vi "DrawSubMenuItems.vi"(7 "Collection in":refnum<class "Collection.lvclass">, 8 "error in (no error)":errorcluster, 9 "Coords":T2, 10 "Tag":string, 11 "Menu in":refnum<class "Menu.lvclass">) -> (0 "error out":errorcluster, 1 "SubMenu":bool, 2 "SelectedArea":T1, 3 "Menu out":refnum<class "Menu.lvclass">, 4 "SelectedItemTag":string, 5 "Collection out":refnum<class "Collection.lvclass">, 6 "GlobalArea":T1)   [LabVIEW 2021, in "Menu.lvlib" / "Menu.lvclass"]
uses:
  Menu.lvclass
  <vilib>/Utility/miscctls.llb/LVPoint32TypeDef.ctl
  Picture2D/src/Collection/Collection.lvclass
  C:/GitHub/Picture2D/src/IDrawable/IDrawable.lvclass
  Picture2D/src/Text/Text.lvclass
  C:/GitHub/Picture2D/src/Picture2D/Picture2D.lvclass
  C:/GitHub/Picture2D/src/Shape/Shape.lvclass
  Picture2D/src/Rectangle/Rectangle.lvclass
  C:/GitHub/Picture2D/src/Polygone/Polygone.lvclass
  Picture2D/src/Point/Point.lvclass
  Picture2D/src/PointSpecialized/PointSpecialized.lvclass
  C:/GitHub/Picture2D/src/Point/Point.lvclass
  Picture2D/src/PointSpecialized/PointSpecialized.lvclass/PointSpecialized.ctl
  Picture2D/src/PointSpecialized/SetColor.vi
  Picture2D/src/Picture/Image.lvclass
  GetFont.vi
  GetDesiredFont.vi
  Picture2D/src/Font/Font.lvclass
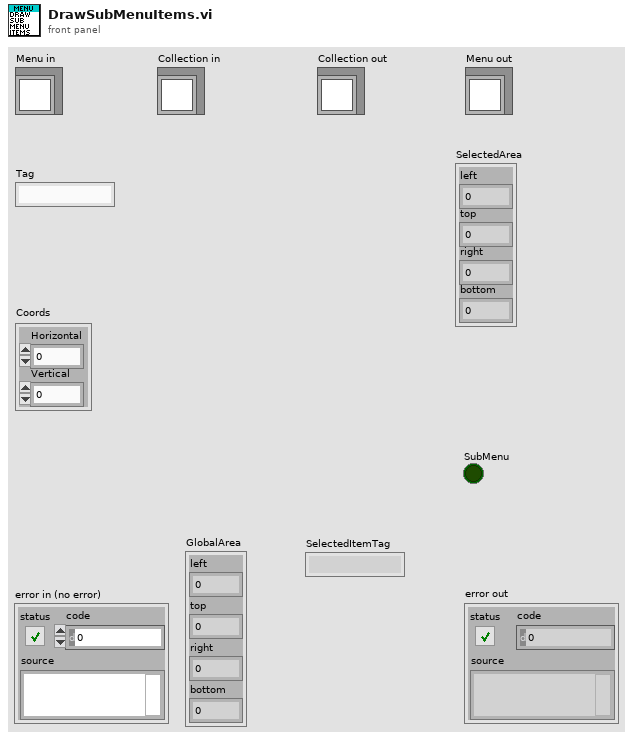
[diagram p1: front panel]
types:
  T1 = cluster{"left":i16, "top":i16, "right":i16, "bottom":i16}
  T2 = typedef "LVPoint32TypeDef.ctl" = cluster{"Horizontal":i32, "Vertical":i32}
  T3 = typedef "Menu.lvlib/Menu.lvclass/MenuItems.ctl" = cluster{"Item Name":string, "Short Cut":T4, "Checked":bool, "Enable":bool, "After item":string, "Item Tags":string[], "Item Names":string[], "Picture":refnum<class "Image.lvclass">, "Hilite Picture":refnum<class "Image.lvclass">, "Displayed":bool}
  T4 = typedef "LVMenuShortCut.ctl" = cluster{"Include Shift Key?":bool, "Include Ctrl Key?":bool, "Shortcut Key":string}
  T5 = typedef "Menu.lvlib/Menu.lvclass/MenuColors.ctl" = cluster{"Text":refnum<class "Color.lvclass">, "HiliteText":refnum<class "Color.lvclass">, "Background":refnum<class "Color.lvclass">, "BorderColor":refnum<class "Color.lvclass">, "Hilite":refnum<class "Color.lvclass">}
  T6 = enum16{"User-specified Font", "Application Font", "System Font", "Dialog Font"}
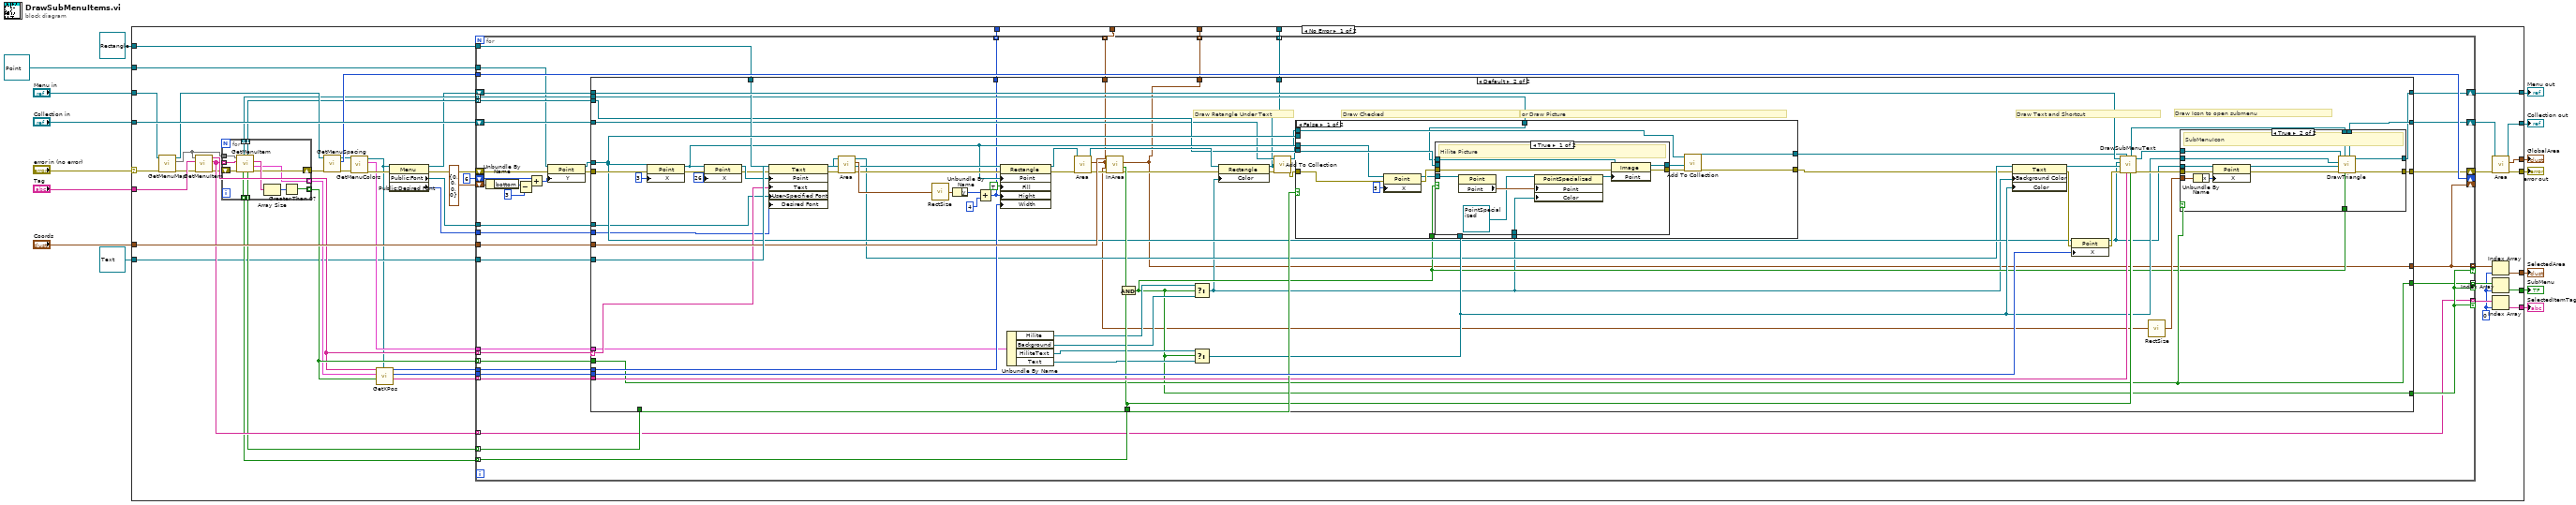
[diagram p0: block diagram]
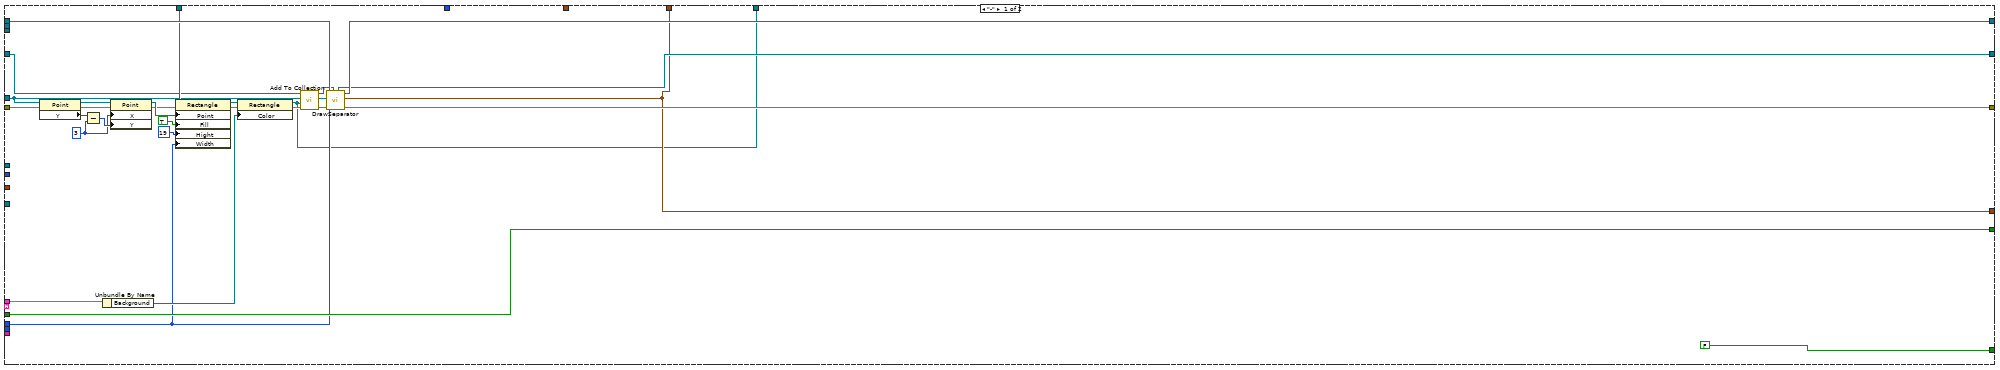
[diagram p2: hidden frame]
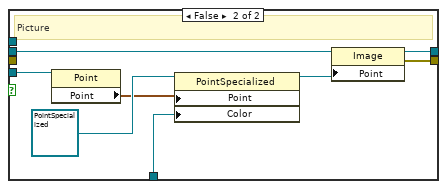
[diagram p3: hidden frame]
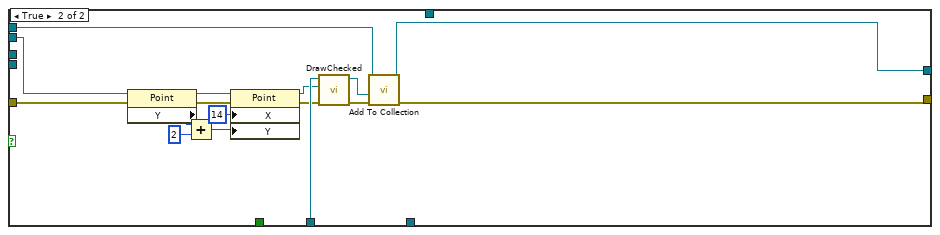
[diagram p4: hidden frame]
diagram:
  n1 = case shown="No Error" "error in (no error)" {
    selector: "error in (no error)" -> [w49 w279]
    tunnel: [w68 _] -> w15
    tunnel: [w66 _] -> w14
    tunnel: "Coords" -> [w62 _]
    tunnel: [w34 _] -> w12
    tunnel: [w55 _] -> w11
    tunnel: "Collection in" -> [w53 w280]
    tunnel: [w29 w280] -> w9
    tunnel: "Menu in" -> [w51 w281]
    tunnel: "Tag" -> [w47 _]
    tunnel: [w40 w279] -> w5
    tunnel: [w30 w281] -> w4
    tunnel: refnum<class "Text.lvclass"> refnum ("Picture2D.lvlib:Text") -> [w27 _]
    tunnel: refnum<class "Point.lvclass"> refnum ("PointSpecialized") -> [w26 _]
    tunnel: refnum<class "Rectangle.lvclass"> refnum ("Rectangle") -> [w25 _]
    tunnel: [w19 _] -> _
    tunnel: [w18 _] -> _
    tunnel: [w17 _] -> _
    tunnel: [w16 _] -> _
    frame No Error {
      w56 = 0 ("index")
      n2 = call "GetMenuMap.vi"("error in (no error)"=w49, "Menu in"=w51) -> ("error out"=w44:errorcluster, "MenuMap"=w48:map{string, T3}, "Menu out"=w50:refnum<class "Menu.lvclass">)  [unwired: 7 in]
      n3 = call "GetMenuItem.vi"("error in (no error)"=w44, "Tag"=w47, "MenuMap"=w48) -> ("error out"=w43:errorcluster, "Item Tags"=w45:string[], "Item Names"=w46:string[])  [unwired: 1 in, 5 out]
      n4 = for {
        tunnel: w48 -> [w278]
        tunnel: w45 -> [w277] mode=indexing
        tunnel: [w274] -> w54 mode=indexing
        shift-right: [w272] -> w42
        shift-left: w43 -> [w273]
        tunnel: [w271] -> w39 mode=indexing
        tunnel: [w270] -> w38 mode=indexing
        tunnel: [w269] -> w37 mode=indexing
        tunnel: [w268] -> w36 mode=indexing
        tunnel: [w267] -> w35 mode=indexing
        n5 = call "GetMenuItem.vi"("error in (no error)"=w273, "Tag"=w277, "MenuMap"=w278) -> ("error out"=w272:errorcluster, "Short Cut"=w271:T4, "Item Tags"=w276:string[], "Checked"=w270:bool, "Picture"=w268:refnum<class "Image.lvclass">, "Enable"=w269:bool, "Hilite Picture"=w267:refnum<class "Image.lvclass">)  [unwired: 1 in, 1 out]
        n6 = Array Size(array=w276) -> (size(s)=w275:i32)
        n7 = Greater Than 0?(x=w275) -> (x > 0?=w274:bool)
      }
      n8 = call "GetMenuSpacing.vi"("error in (no error)"=w42, "Menu in"=w50) -> ("error out"=w41:errorcluster, "MenuSpacing"=w52:i32, "Menu out"=w33:refnum<class "Menu.lvclass">)  [unwired: 7 in]
      n9 = call "GetMenuColors.vi"("error in (no error)"=w41, "Menu in"=w33) -> ("error out"=w31:errorcluster, "MenuColors"=w28:T5, "Menu out"=w20:refnum<class "Menu.lvclass">)  [unwired: 7 in]
      n10 = call "GetXPos.vi"("Menu"=w20, "SubMenu"=w54, "Array"=w39, "Item Names"=w46) -> ("ShortCut Text"=w59:string[], "Start ShortCut"=w60:i16, "Total X"=w61:i16)  [unwired: 5 in]
      n11 = property class="Menu"(reference=w20, error in=w31) -> (reference out=w23:refnum<class "Menu.lvclass">, error out=w24:errorcluster, "Public:Font"=w22:refnum<class "Font.lvclass">, "Public:Desired Font"=w21:T6)
      n12 = for {
        tunnel: w46 -> [w101] mode=indexing
        shift-right: [w98] -> w58
        shift-left: w53 -> [w99]
        shift-right: [w100] -> _
        shift-left: T1 {"left"=0, "top"=0, "right"=0, "bottom"=0} ("Area out") -> [w106]
        tunnel: w62 -> [w103]
        shift-right: [w102] -> _
        shift-left: i16 6 ("Spacing") -> [w104]
        tunnel: w52 -> [w102]
        tunnel: [w83] -> w65 mode=indexing if=w93
        tunnel: [w100] -> w67 mode=indexing if=w93
        tunnel: w45 -> [w83] mode=indexing
        tunnel: w61 -> [w97]
        tunnel: w60 -> [w96]
        tunnel: w59 -> [w95] mode=indexing
        tunnel: w54 -> [w94] mode=indexing
        tunnel: [w84] -> w57 mode=indexing if=w93
        tunnel: w38 -> [w90] mode=indexing
        tunnel: w37 -> [w85] mode=indexing
        tunnel: w36 -> [w91] mode=indexing
        tunnel: w35 -> [w89] mode=indexing
        shift-right: [w88] -> w32
        shift-left: w24 -> [w87]
        shift-right: [w76] -> w30
        shift-left: w23 -> [w86]
        tunnel: w28 -> [w82]
        tunnel: w27 -> [w81]
        tunnel: w26 -> [w80]
        tunnel: w25 -> [w79]
        tunnel: w22 -> [w78]
        tunnel: w21 -> [w77]
        tunnel: [w75] -> w19 mode=indexing
        tunnel: [w74] -> w18 mode=indexing
        tunnel: [w73] -> w17 mode=indexing
        tunnel: [w72] -> w16 mode=indexing
        n13 = Unbundle By Name(w106) -> ("bottom"=w71:i16)
        n14 = Subtract(x=w71, y=i16 3) -> (x-y=w70:i16)
        n15 = Add(x=w104, y=w70) -> (x+y=w105:i32)
        n16 = property class="Point"(reference=w80, error in=w87, "Y"=w105) -> (reference out=w107:refnum<class "Point.lvclass">, error out=w92:errorcluster)
        n17 = case shown="Default" w101 {
          selector: w101 -> [_ w195]
          tunnel: w107 -> [w119 w173]
          tunnel: w103 -> [_ w198]
          tunnel: w81 -> [_ w203]
          tunnel: [w109 w138] -> w100
          tunnel: [FALSE ("InArea") w150] -> w93
          tunnel: w99 -> [w122 w145]
          tunnel: [w110 w158] -> w98
          tunnel: w97 -> [w123 w196]
          tunnel: w96 -> [_ w194]
          tunnel: w95 -> [_ w182]
          tunnel: w94 -> [w135 w180]
          tunnel: [w135 w180] -> w84
          tunnel: w92 -> [w111 w192]
          tunnel: w91 -> [_ w149]
          tunnel: w90 -> [_ w187]
          tunnel: w89 -> [_ w148]
          tunnel: [w134 w177] -> w88
          tunnel: w86 -> [w133 w184]
          tunnel: w85 -> [_ w181]
          tunnel: w82 -> [w126 w172]
          tunnel: w79 -> [w124 w167]
          tunnel: w78 -> [_ w156]
          tunnel: w77 -> [_ w162]
          tunnel: [w132 w157] -> w76
          tunnel: [_ w140] -> w75
          tunnel: [w109 w138] -> w74
          tunnel: [_ w139] -> w73
          tunnel: [w108 w137] -> w72
          frame "-" {
            w115 = i16 3 ("Point:x")
            n18 = property class="Point"(reference=w119, error in=w111) -> (reference out=w116:refnum<class "Point.lvclass">, error out=w114:errorcluster, "Y"=w118:i16)
            n19 = Subtract(x=w118, y=w115) -> (x-y=w117:i16)
            n20 = Unbundle By Name(w126) -> ("Background"=w125:refnum<class "Color.lvclass">)
            n21 = property class="Point"(reference=w116, error in=w114, "X"=w115, "Y"=w117) -> (reference out=w120:refnum<class "Point.lvclass">, error out=w113:errorcluster)
            n22 = property class="Rectangle"(reference=w124, error in=w113, "Point"=w120, "Fill"=TRUE, "Hight"=i16 19 ("x"), "Width"=w123) -> (reference out=w128:refnum<class "Rectangle.lvclass">, error out=w130:errorcluster)
            n23 = property class="Rectangle"(reference=w128, error in=w130, "Color"=w125) -> (reference out=w108:refnum<class "Rectangle.lvclass">, error out=w129:errorcluster)
            n24 = call-dynamic "Add To Collection.vi"("error in (no error)"=w129, "IDrawable"=w108, "Collection in"=w122) -> ("error out"=w112:errorcluster, "Collection out"=w121:refnum<class "Collection.lvclass">)  [unwired: 7 in]
            n25 = call "DrawSeparator.vi"("Collection in"=w121, "error in (no error)"=w112, "XPos"=w123, "Point"=w119, "Menu in"=w133) -> ("error out"=w134:errorcluster, "rect"=w109:T1, "Menu out"=w132:refnum<class "Menu.lvclass">, "Collection out"=w110:refnum<class "Collection.lvclass">)  [unwired: 3 in]
          }
          frame Default {
            # "Draw Retangle Under Text"
            # "Draw Checked"
            # "or Draw Picture"
            # "Draw Icon to open submenu"
            # "Draw Text and Shortcut"
            n26 = property class="Point"(reference=w173, error in=w192, "X"=i16 3 ("Point:x")) -> (reference out=w151:refnum<class "Point.lvclass">, error out=w166:errorcluster)
            n27 = property class="Point"(reference=w151, error in=w166, "X"=i16 26 ("Point:x")) -> (reference out=w202:refnum<class "Point.lvclass">, error out=w165:errorcluster)
            n28 = property class="Text"(reference=w203, error in=w165, "Point"=w202, "Text"=w195, "User-Specified Font"=w156, "Desired Font"=w162) -> (reference out=w155:refnum<class "Text.lvclass">, error out=w191:errorcluster)
            n29 = call-dynamic "Area.vi"("error in (no error)"=w191, "Text in"=w155) -> ("error out"=w190:errorcluster, "rect"=w197:T1, "Text out"=w154:refnum<class "Text.lvclass">)  [unwired: 7 in]
            n30 = call <vilib>:"RectSize.vi"("rect"=w197) -> ("point"=w199:cluster{"x":i16, "y":i16})
            n31 = Unbundle By Name(w199) -> ("y"=w153:i16)
            n32 = Add(x=w153, y=i16 4) -> (x+y=w140:i16)
            n33 = property class="Rectangle"(reference=w167, error in=w190, "Point"=w151, "Fill"=TRUE, "Hight"=w140, "Width"=w196) -> (reference out=w164:refnum<class "Rectangle.lvclass">, error out=w189:errorcluster)
            n34 = Unbundle By Name(w172) -> ("Hilite"=w168:refnum<class "Color.lvclass">, "Background"=w169:refnum<class "Color.lvclass">, "HiliteText"=w171:refnum<class "Color.lvclass">, "Text"=w170:refnum<class "Color.lvclass">)
            n35 = call-dynamic "Area.vi"("error in (no error)"=w189, "Rectangle in"=w164) -> ("error out"=w188:errorcluster, "rect"=w139:T1, "Rectangle out"=w163:refnum<class "Rectangle.lvclass">)  [unwired: 7 in]
            n36 = call "InArea.vi"("error in (no error)"=w188, "Area in"=w139, "Coords"=w198) -> ("error out"=w146:errorcluster, "InArea"=w186:bool, "Area out"=w138:T1)  [unwired: 6 in]
            n37 = Compound Arithmetic op=AND(w186, w181) -> (w150:bool)
            n38 = Select(t=w168, s=w150, f=w169) -> (s? t:f=w147:refnum<class "Color.lvclass">)
            n39 = Select(t=w171, s=w150, f=w170) -> (s? t:f=w174:refnum<class "Color.lvclass">)
            n40 = property class="Rectangle"(reference=w163, error in=w146, "Color"=w147) -> (reference out=w137:refnum<class "Rectangle.lvclass">, error out=w185:errorcluster)
            n41 = call-dynamic "Add To Collection.vi"("error in (no error)"=w185, "IDrawable"=w137, "Collection in"=w145) -> ("error out"=w142:errorcluster, "Collection out"=w144:refnum<class "Collection.lvclass">)  [unwired: 7 in]
            n42 = case shown="False" w187 {
              tunnel: w144 -> [w211 w250]
              tunnel: w142 -> [w213 w239]
              tunnel: w174 -> [_ w249]
              tunnel: w173 -> [_ w237]
              tunnel: w151 -> [w204 _]
              tunnel: w150 -> [w210 _]
              tunnel: w149 -> [w209 _]
              tunnel: w148 -> [w208 _]
              tunnel: w147 -> [w207 _]
              tunnel: [w205 w235] -> w141
              tunnel: [w206 w236] -> w143
              frame False {
                n43 = property class="Point"(reference=w204, error in=w213, "X"=i16 5 ("Point:x")) -> (reference out=w215:refnum<class "Point.lvclass">, error out=w217:errorcluster)
                n44 = case shown="True" w210 {
                  tunnel: w209 -> [_ w233]
                  tunnel: [w226 w234] -> w214
                  tunnel: w215 -> [w221 w231]
                  tunnel: w208 -> [w225 _]
                  tunnel: [w224 w232] -> w216
                  tunnel: w217 -> [w223 _]
                  tunnel: w207 -> [w218 w227]
                  frame True {
                    # "Hilite Picture"
                    n45 = property class="Point"(reference=w221) -> ("Point"=w222:cluster{"x":i16, "y":i16})  [unwired: 1 in, 2 out]
                    n46 = property class="PointSpecialized"(reference=refnum<class "PointSpecialized.lvclass"> refnum ("Picture2D.lvlib:PointSpecialized"), "Point"=w222, "Color"=w218) -> (reference out=w220:refnum<class "PointSpecialized.lvclass">)  [unwired: 1 in, 1 out]
                    n47 = property class="Image"(reference=w225, error in=w223, "Point"=w220) -> (reference out=w226:refnum<class "Image.lvclass">, error out=w224:errorcluster)
                  }
                  frame False {
                    # "Picture"
                    n48 = property class="Point"(reference=w231) -> ("Point"=w229:cluster{"x":i16, "y":i16})  [unwired: 1 in, 2 out]
                    n49 = property class="PointSpecialized"(reference=refnum<class "PointSpecialized.lvclass"> refnum ("Picture2D.lvlib:PointSpecialized"), "Point"=w229, "Color"=w227) -> (reference out=w228:refnum<class "PointSpecialized.lvclass">)  [unwired: 1 in, 1 out]
                    n50 = property class="Image"(reference=w233, "Point"=w228) -> (reference out=w234:refnum<class "Image.lvclass">, error out=w232:errorcluster)  [unwired: 1 in]
                  }
                }
                n51 = call-dynamic "Add To Collection.vi"("error in (no error)"=w216, "IDrawable"=w214, "Collection in"=w211) -> ("error out"=w205:errorcluster, "Collection out"=w206:refnum<class "Collection.lvclass">)  [unwired: 7 in]
              }
              frame True {
                n52 = property class="Point"(reference=w237, error in=w239) -> (reference out=w245:refnum<class "Point.lvclass">, error out=w238:errorcluster, "Y"=w246:i16)
                n53 = Add(x=w246, y=i16 2) -> (x+y=w247:i16)
                n54 = property class="Point"(reference=w245, error in=w238, "X"=i16 14 ("Point:x"), "Y"=w247) -> (reference out=w242:refnum<class "Point.lvclass">, error out=w241:errorcluster)
                n55 = call "DrawChecked.vi"("error in"=w241, "Point"=w242, "Color"=w249) -> ("error out"=w240:errorcluster, "Collection out"=w248:refnum<class "Collection.lvclass">)  [unwired: 7 in]
                n56 = call-dynamic "Add To Collection.vi"("error in (no error)"=w240, "IDrawable"=w248, "Collection in"=w250) -> ("error out"=w235:errorcluster, "Collection out"=w236:refnum<class "Collection.lvclass">)  [unwired: 7 in]
              }
            }
            n57 = property class="Text"(reference=w154, error in=w141, "Background Color"=w147, "Color"=w174) -> (reference out=w183:refnum<class "Text.lvclass">, error out=w176:errorcluster)
            n58 = property class="Point"(reference=w173, error in=w176, "X"=w194) -> (reference out=w160:refnum<class "Point.lvclass">, error out=w175:errorcluster)
            n59 = call "DrawSubMenuText.vi"("Enable"=w181, "ShortcutText"=w182, "Collection in"=w143, "error in (no error)"=w175, "Text"=w183, "InsertionPoint"=w160, "Menu in"=w184) -> ("error out"=w178:errorcluster, "Menu out"=w161:refnum<class "Menu.lvclass">, "Collection out"=w159:refnum<class "Collection.lvclass">)  [unwired: 2 in]
            n60 = call <vilib>:"RectSize.vi"("rect"=w139) -> ("point"=w179:cluster{"x":i16, "y":i16})
            n61 = case shown="True" w180 {
              tunnel: w174 -> [_ w256]
              tunnel: [w253 w262] -> w177
              tunnel: w179 -> [_ w265]
              tunnel: w160 -> [_ w264]
              tunnel: w178 -> [w253 w263]
              tunnel: w161 -> [w251 w257]
              tunnel: w150 -> [_ w258]
              tunnel: w159 -> [w252 w260]
              tunnel: [w252 w259] -> w158
              tunnel: [w251 w254] -> w157
              frame False {
                # "No Triangle"
              }
              frame True {
                # "SubMenuIcon"
                n62 = Unbundle By Name(w265) -> ("x"=w266:i16)
                n63 = property class="Point"(reference=w264, error in=w263, "X"=w266) -> (reference out=w255:refnum<class "Point.lvclass">, error out=w261:errorcluster)
                n64 = call "DrawTriangle.vi"("Open?"=w258, "Collection in"=w260, "error in"=w261, "Point"=w255, "Color"=w256, "Menu in"=w257) -> ("error out"=w262:errorcluster, "Menu out"=w254:refnum<class "Menu.lvclass">, "Collection out"=w259:refnum<class "Collection.lvclass">)  [unwired: 3 in]
              }
            }
          }
        }
      }
      n65 = call-dynamic "Area.vi"("error in (no error)"=w32, "Collection in"=w58) -> ("error out"=w40:errorcluster, "Area"=w34:T1, "Collection out"=w29:refnum<class "Collection.lvclass">)  [unwired: 7 in]
      n66 = Index Array(array=w67, index=w56) -> (element=w68:T1)
      n67 = Index Array(array=w57, index=w56) -> (element=w55:bool)
      n68 = Index Array(array=w65, index=w56) -> (element=w66:string)
    }
    frame Error {
    }
  }
  "error out" <- w5
  "Menu out" <- w4
  "SelectedArea" <- w15
  "SelectedItemTag" <- w14
  "GlobalArea" <- w12
  "SubMenu" <- w11
  "Collection out" <- w9
